vi "Init.vi"(6 "Filter":T1 {"Deny List (ID)" format="%.0x"; "Allow List (ID)" format="%.0x"}, 8 "error in (no error)":errorcluster, 9 "Port Configuration":T2={"Mode"=enum."CAN FD", "Baud Rate"=500000, "Temination On"=TRUE, "Subordinate"=FALSE, "Echo TX"=FALSE, "FD Config"={"FD Baud Rate"=2000000, "ISO Mode"=TRUE, "BRS Enabled"=TRUE}} {"FD Config"."FD Baud Rate" format="%.0p"; "Baud Rate" format="%.0p"}, 10 "Interface":string, 11 "CAN_RW_CORE in":refnum<class "CAN_RW_CORE.lvclass">) -> (0 "error out":errorcluster, 3 "CAN_RW_CORE out":refnum<class "CAN_RW_CORE.lvclass">)   [LabVIEW 2021, in "CAN_RW_CORE.lvclass"]
uses:
  CAN_RW_CORE.lvclass
  typedef/CAN Port Configuration.ctl
  typedef/CAN Mode.ctl
  typedef/FD Config.ctl
  typedef/CAN Filter.ctl
  typedef/CAN Interface Mode.ctl
  <vilib>/CIF Foundation/CIF PCAP Parse and Build/Typedef/File Format.ctl
  <vilib>/CIF Foundation/CIF Utilities/DataTypes/Typedef/Endian.ctl
  <vilib>/CIF Foundation/CIF PCAP Parse and Build/Typedef/Time Format.ctl
  <vilib>/CIF Foundation/CIF PCAP Parse and Build/pcap_Parse_Build_CIF.lvclass/pcap_Parse_Build_CIF.ctl
  CAN_RW_CORE.lvclass/CAN_RW_CORE.ctl
  <vilib>/CIF Foundation/CIF PCAP Parse and Build/Data Accessors/Write pcap format.vi
  <vilib>/CIF Foundation/CIF PCAP Parse and Build/Data Accessors/Write OS Endian.vi
  <vilib>/CIF Foundation/CIF PCAP Parse and Build/pcap_Parse_Build_CIF.lvclass
  <vilib>/CIF Foundation/CIF Utilities/DataTypes/DataTypes_CIF_U.lvlib
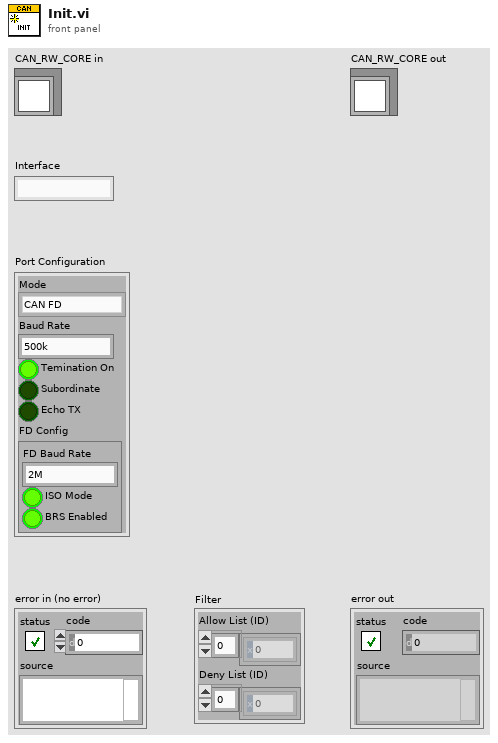
[diagram p1: front panel]
types:
  T1 = typedef "CAN_RW_CORE.lvclass/CAN Filter.ctl" = cluster{"Allow List (ID)":u32[], "Deny List (ID)":u32[]}
  T2 = typedef "CAN_RW_CORE.lvclass/CAN Port Configuration.ctl" = cluster{"Mode":T3, "Baud Rate":u64, "Temination On":bool, "Subordinate":bool, "Echo TX":bool, "FD Config":T4}
  T3 = typedef "CAN_RW_CORE.lvclass/CAN Mode.ctl" = enum16{"CAN 2.0", "CAN FD"}
  T4 = typedef "CAN_RW_CORE.lvclass/FD Config.ctl" = cluster{"FD Baud Rate":u64, "ISO Mode":bool, "BRS Enabled":bool}
  T5 = typedef "DataTypes_CIF_U.lvlib/Endian.ctl" = enum16{"Little Endian", "Big Endian"}
  T6 = typedef "pcap_Parse_Build_CIF.lvclass/File Format.ctl" = cluster{"Endian":T5, "Time Format":T7}
  T7 = typedef "pcap_Parse_Build_CIF.lvclass/Time Format.ctl" = enum16{"us", "ns"}
  T8 = typedef "CAN_RW_CORE.lvclass/CAN Interface Mode.ctl" = enum16{"Unknown", "CAN 2.0", "CAN FD", "CAN FD BRS"}
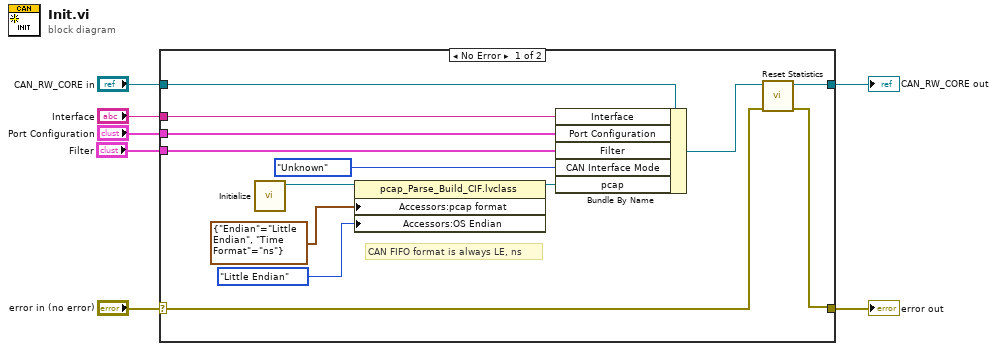
[diagram p0: block diagram]
diagram:
  n1 = case shown="No Error" "error in (no error)" {
    selector: "error in (no error)" -> [w13 w22]
    tunnel: [w12 w22] -> w6
    tunnel: [w14 w21] -> w4
    tunnel: "CAN_RW_CORE in" -> [w20 w21]
    tunnel: "Interface" -> [w19 _]
    tunnel: "Port Configuration" -> [w18 _]
    tunnel: "Filter" -> [w17 _]
    frame No Error {
      # "CAN FIFO format is always LE, ns"
      n2 = call <vilib>:"Initialize.vi"() -> ("pcap Parse and Build out"=w10:refnum<class "pcap_Parse_Build_CIF.lvclass">)  [unwired: 11 in]
      n3 = property class="pcap_Parse_Build_CIF.lvclass"(reference=w10, "Accessors:pcap format"=T6 {"Endian"=enum."Little Endian", "Time Format"=enum."ns"} ("pcap format"), "Accessors:OS Endian"=Endian."Little Endian" ("OS Endian")) -> (reference out=w9:refnum<class "pcap_Parse_Build_CIF.lvclass">)  [unwired: 1 in, 1 out]
      n4 = Bundle By Name(cluster=w20, "Interface"=w19, "Port Configuration"=w18, "Filter"=w17, "CAN Interface Mode"=CAN_Interface_Mode."Unknown", "pcap"=w9) -> (w15:refnum<class "CAN_RW_CORE.lvclass">)
      n5 = call "Reset Statistics.vi"("error in (no error)"=w13, "CAN_RW_CORE in"=w15) -> ("error out"=w12:errorcluster, "CAN_RW_CORE out"=w14:refnum<class "CAN_RW_CORE.lvclass">)  [unwired: 8 in]
    }
    frame Error {
    }
  }
  "error out" <- w6
  "CAN_RW_CORE out" <- w4
